vi "pvdf_forcereconstructor.vi"() -> ()   [LabVIEW 2023]
uses:
  MessageType.ctl
  <vilib>/Instr/_visa.llb/VISA Configure Serial Port (Instr).vi
panel:
  in  "?":enum32{"PVDF Plot", "Force Plot", "Heatmap"}(tab)
  out "Sensors data":T1(graph)
  out "Reconstructed force":T1(graph)
  out "Index":T2={"S2"=655360, "S3"=655360, "S6"=655360, "S7 3"=655360, "S8 4"=655360, "S4 2"=655360, "S1"=655360, "S5"=655360}
  out "Thumb":T2
  in  "?":T3(tab)
  in  "Header":string="<>\u0000"
  in  "Alpha":dbl=1.0 min=0.0 max=1.0
  out "READ BUFFER":string
  in  "COM_IE":refnum<visa-resource-name>="COM3"
  in  "Commands":string[](array[string])
  out "Error Out":errorcluster
  in  "Number of sensors":u32=16
  in  "block size":u32=100
  in  "PVDF Folder to Save":string="pvdf_data"
  in  "PVDF File Name Root":string="pvdf"
  out "Resulting pvdf saving path":path
  in  "Save pvdf only":bool
  in  "PVDF and Force Folder to Save":string="pvdf_force_data"
  in  "PVDF and Force File Name Root":string="pvdf_force"
  out "Resulting pvdf and force saving path":path
  in  "Save pvdf and force":bool
  in  "Active channels":bool[][](array[boolean])
  out "bytes to read":u32
  in  "TCP cluster":cluster{"data":dbl[][], "timestamp":u32[]}
  in  "pvdf and force save cluster":cluster{"Controls":T4, "data":string}
  in  "pvdf plot cluster":T1
  in  "pvdf save cluster":cluster{"Controls":T4, "data":string}
  in  "Stop":bool
  # "1"
  # "0.5"
  # "0"
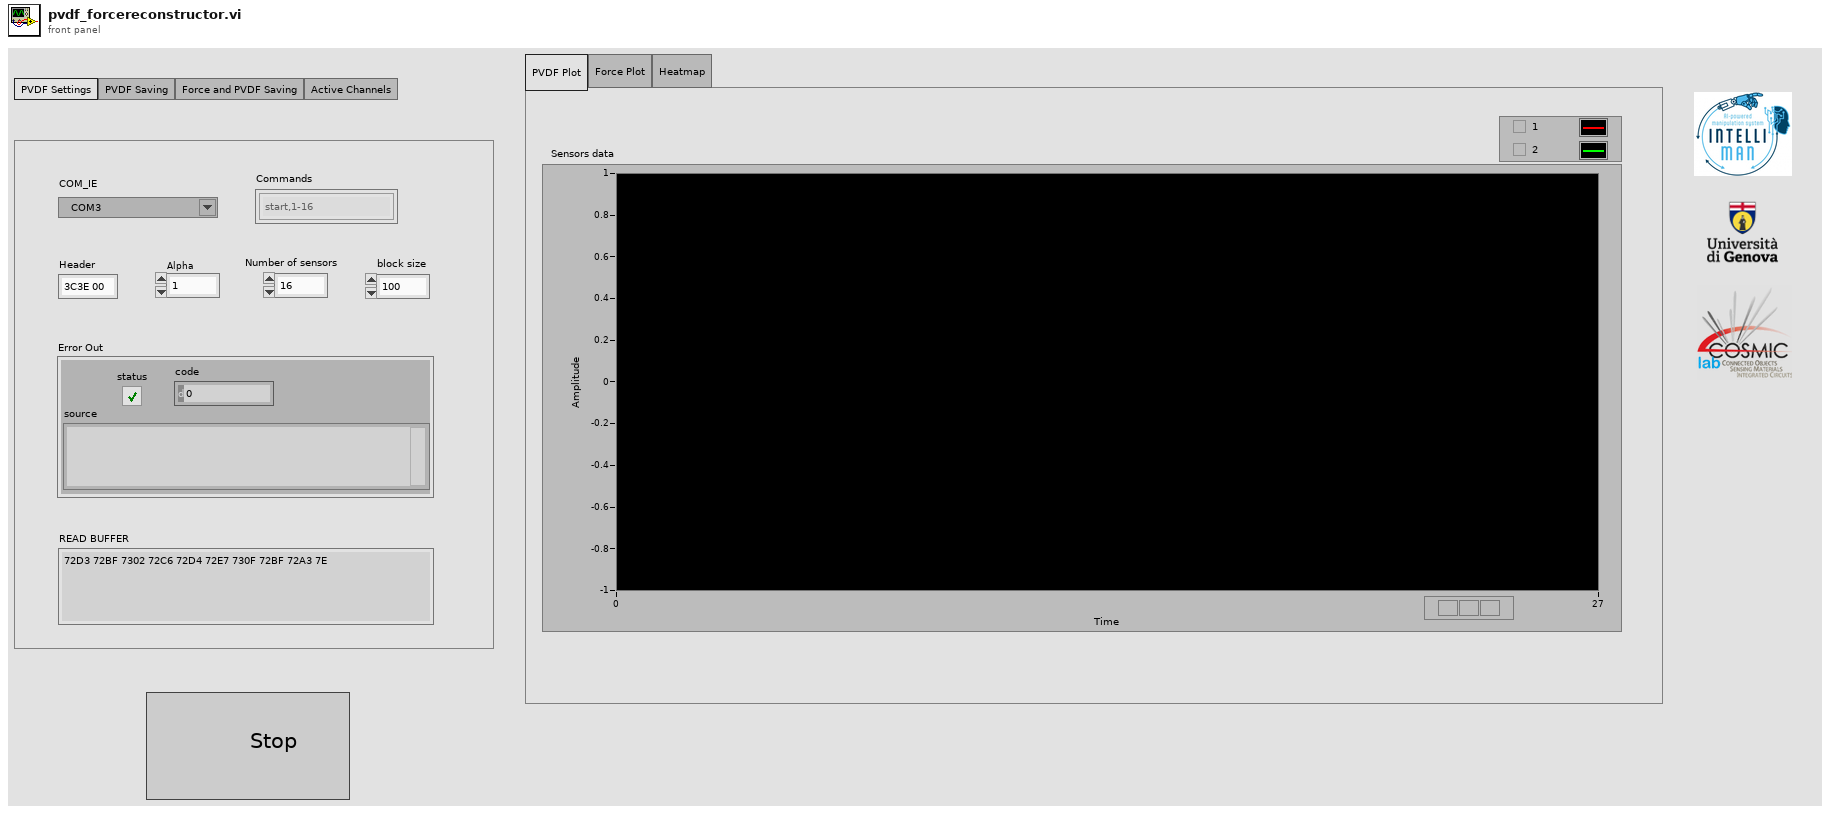
[diagram p1: front panel]
types:
  T1 = cluster{"[0]":dbl, "[1]":dbl, "[2]":dbl, "[3]":dbl, "[4]":dbl, "[5]":dbl, "[6]":dbl, "[7]":dbl, "[8]":dbl, "[9]":dbl, "[10]":dbl, "[11]":dbl, "[12]":dbl, "[13]":dbl, "[14]":dbl, "[15]":dbl, "[16]":dbl, "[17]":dbl, "[18]":dbl, "[19]":dbl, "[20]":dbl, "[21]":dbl, "[22]":dbl, "[23]":dbl, "[24]":dbl, "[25]":dbl, "[26]":dbl, "[27]":dbl, "[28]":dbl, "[29]":dbl, "[30]":dbl, "[31]":dbl, "[32]":dbl, "[33]":dbl, "[34]":dbl, "[35]":dbl, "[36]":dbl, "[37]":dbl, "[38]":dbl, "[39]":dbl, "[40]":dbl, "[41]":dbl, "[42]":dbl, "[43]":dbl, "[44]":dbl, "[45]":dbl, "[46]":dbl, "[47]":dbl, "[48]":dbl, "[49]":dbl, "[50]":dbl, "[51]":dbl, "[52]":dbl, "[53]":dbl, "[54]":dbl, "[55]":dbl, "[56]":dbl, "[57]":dbl, "[58]":dbl, "[59]":dbl, "[60]":dbl, "[61]":dbl, "[62]":dbl, "[63]":dbl}
  T2 = cluster{"S2":u32, "S3":u32, "S6":u32, "S7 3":u32, "S8 4":u32, "S4 2":u32, "S1":u32, "S5":u32}
  T3 = enum32{"PVDF Settings", "PVDF Saving", "Force and PVDF Saving", "Active Channels"}
  T4 = typedef "MessageType.ctl" = enum16{"data", "start_save", "stop_save", "active_channels"}
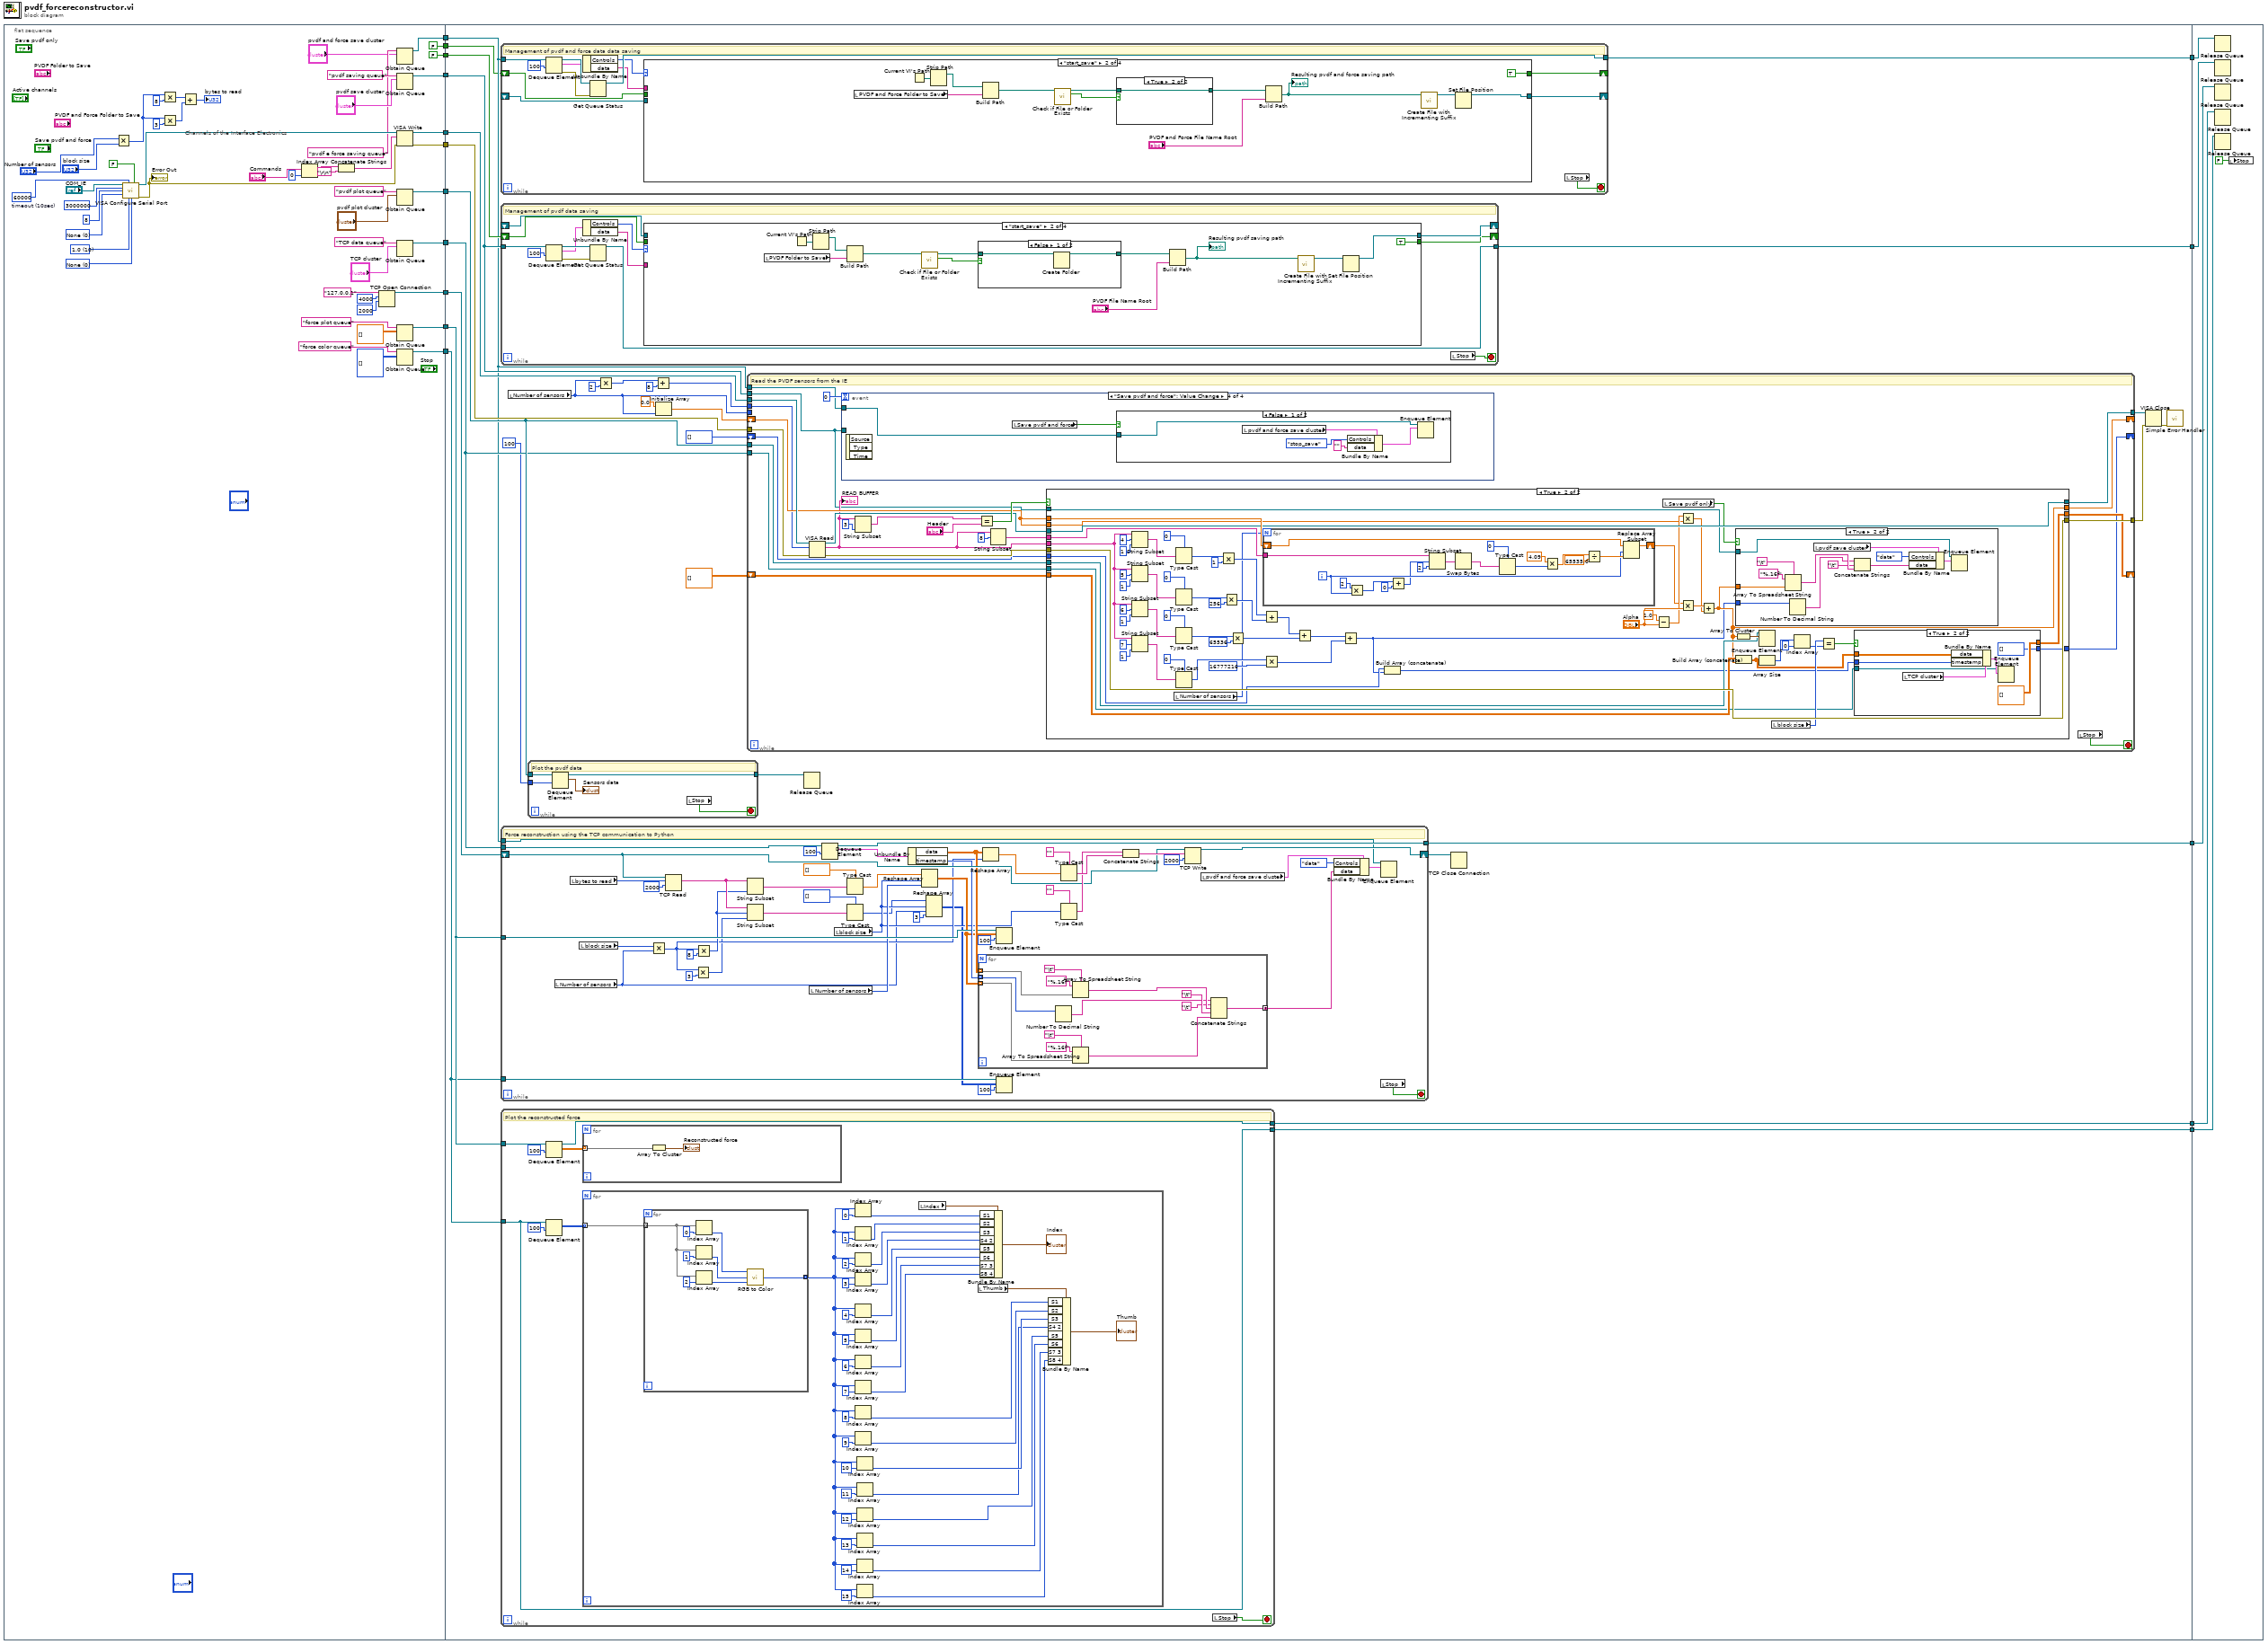
[diagram p0: block diagram]
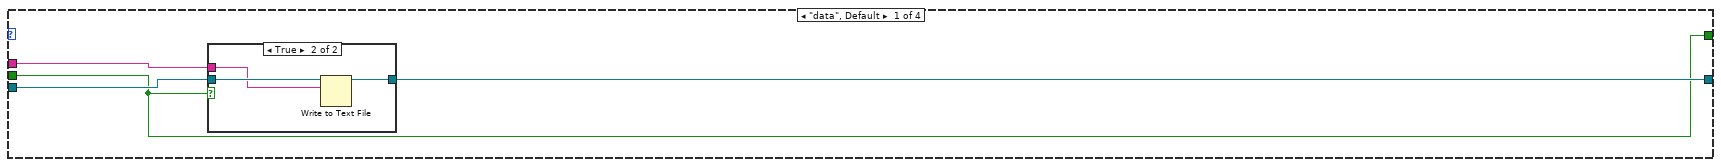
[diagram p2: hidden frame]
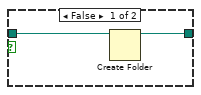
[diagram p4: hidden frame]
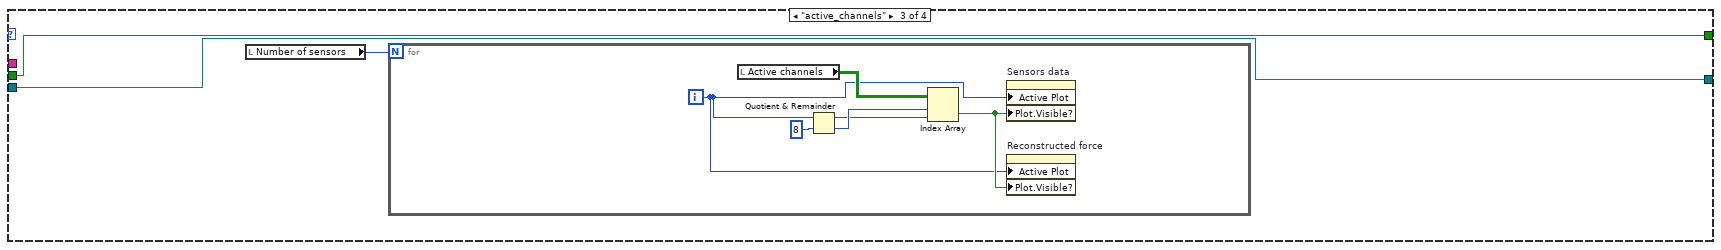
[diagram p5: hidden frame]
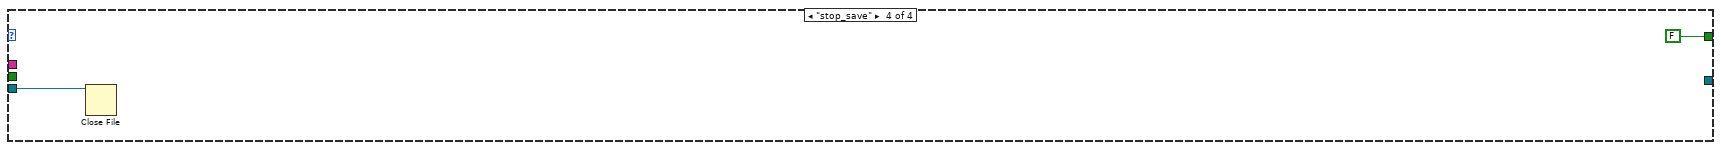
[diagram p6: hidden frame]
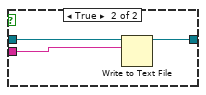
[diagram p8: hidden frame]
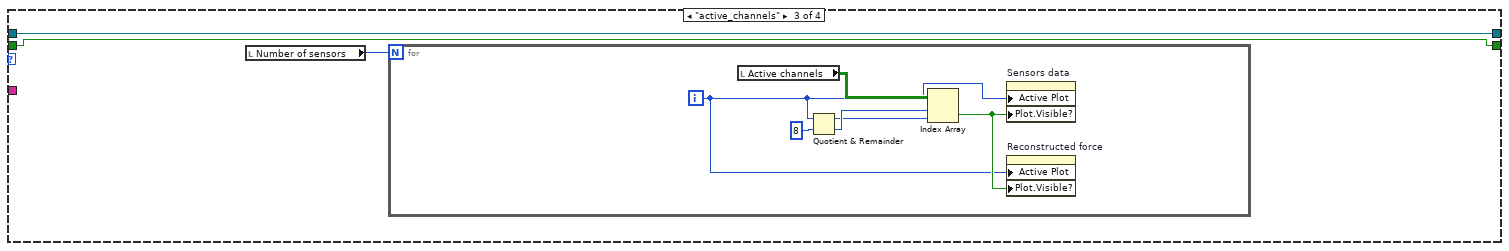
[diagram p10: hidden frame]
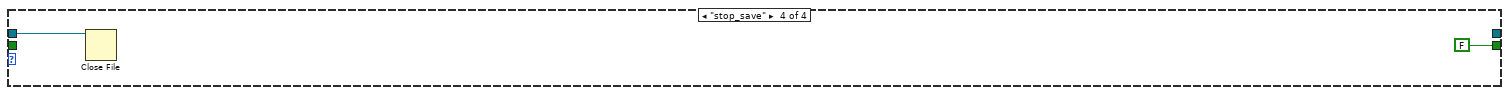
[diagram p11: hidden frame]
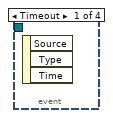
[diagram p12: hidden frame]
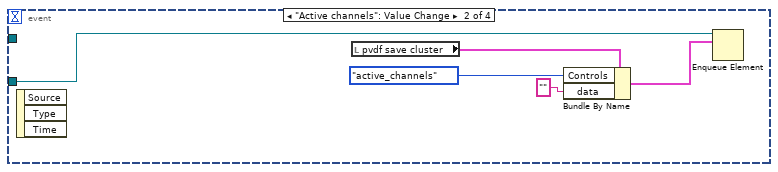
[diagram p13: hidden frame]
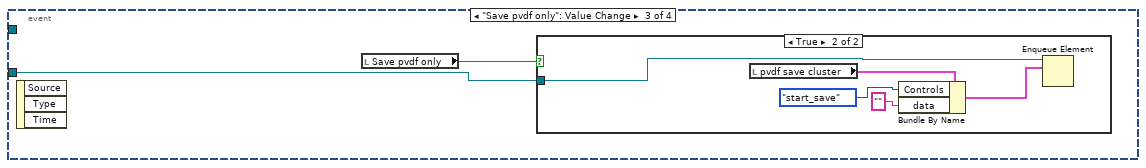
[diagram p14: hidden frame]
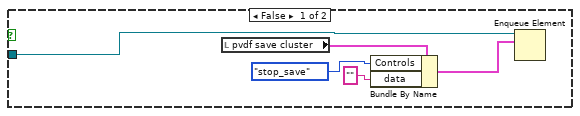
[diagram p15: hidden frame]
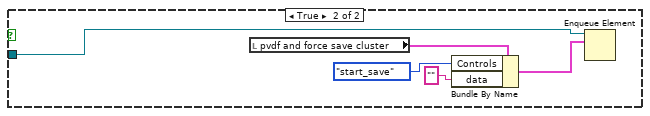
[diagram p16: hidden frame]
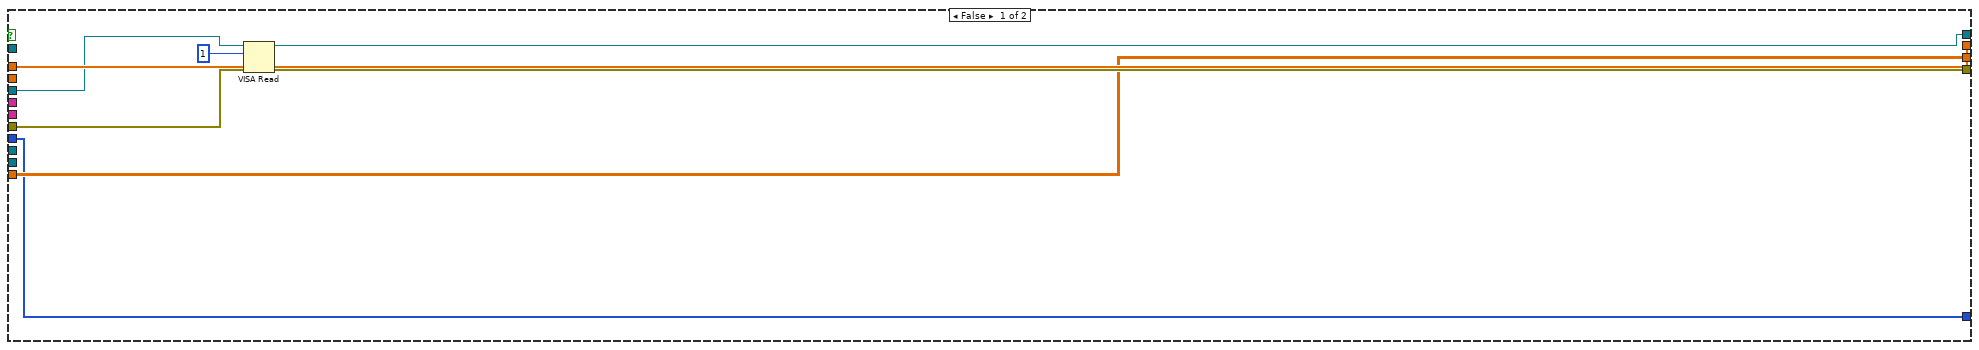
[diagram p17: hidden frame]
diagram:
  n1 = flat-sequence {
    tunnel: [w63] -> w16
    tunnel: [FALSE ("start save pvdf")] -> w15
    tunnel: [w60] -> w14
    tunnel: [w44] -> w13
    tunnel: [w43] -> w12
    tunnel: [w41] -> w11
    tunnel: [w38] -> w10
    tunnel: [w35] -> w9
    tunnel: [FALSE ("start save pvdf and force")] -> w8
    tunnel: [w29] -> w7
    tunnel: [w19] -> w6
    tunnel: w16 -> [w87]
    tunnel: w15 -> [w86]
    tunnel: w14 -> [w85]
    tunnel: w13 -> [w83]
    tunnel: w12 -> [w84]
    tunnel: w11 -> [w80]
    tunnel: w10 -> [w78]
    tunnel: w9 -> [w77]
    tunnel: w8 -> [w76]
    tunnel: w7 -> [w74]
    tunnel: w6 -> [w71]
    tunnel: [w70] -> w5
    tunnel: [w69] -> w4
    tunnel: [w68] -> w3
    tunnel: [w67] -> w2
    tunnel: [w66] -> w1
    tunnel: w5 -> [w477]
    tunnel: w4 -> [w476]
    tunnel: w3 -> [w475]
    tunnel: w2 -> [w474]
    tunnel: w1 -> [w473]
    frame #0 {
      w45 = u16 0 items=["None"=0, "XON/XOFF"=1, "RTS/CTS"=2, "DTR/DSR"=4] ("flow control")
      w51 = u32 60000  # timeout (10sec)
      w47 = u16 0 items=["None", "Odd", "Even", "Mark", "Space"] ("parity (0:none)")
      w46 = u16 10 items=["1.0"=10, "1.5"=15, "2.0"=20] ("stop bits")
      # "Channels of the Interface Electronics"
      n2 = Multiply(x="Number of sensors", y="block size") -> (x*y=w24:u32)
      n3 = call-poly "VISA Configure Serial Port"("VISA resource name"="COM_IE", "timeout (10sec)"=w51, "Enable Termination\nChar (T)"=FALSE ("Enable Termination\nChar (T)"), "baud rate (9600)"=u32 3000000, "data bits (8)"=u16 8, "parity (0:none)"=w47, "stop bits (10: 1 bit)"=w46, "flow control (0:none)"=w45) -> ("VISA resource name out"=w55:refnum<visa-resource-name>, "error out"=w56:errorcluster)  [unwired: 6 in]
      "Error Out" <- w56
      n4 = Multiply(x=w24, y=u32 8) -> (x*y=w26:u32)
      n5 = Multiply(x=w24, y=u32 3) -> (x*y=w25:u32)
      n6 = Add(x=w26, y=w25) -> (x+y=→"bytes to read":u32)
      n7 = Index Array(array="Commands", index=0) -> (element=w58:string)
      n8 = Concatenate Strings(w58, "\r\n") -> (w59:string)
      n9 = TCP Open Connection(address="127.0.0.1", remote port or service name=u16 4000, timeout ms (60000)=2000) -> (connection ID=w41:refnum<k5>)  [unwired: 2 in, 1 out]
      n10 = Obtain Queue(name (unnamed)="pvdf e force saving queue", element data type="pvdf and force save cluster") -> (queue out=w35:refnum<queue>)  [unwired: 3 in, 2 out]
      n11 = Obtain Queue(name (unnamed)="pvdf saving queue", element data type="pvdf save cluster") -> (queue out=w63:refnum<queue>)  [unwired: 3 in, 2 out]
      n12 = VISA Write(VISA resource name=w55, write buffer=w59, error in (no error)=w56) -> (VISA resource name out=w43:refnum<visa-resource-name>, error out=w44:errorcluster)  [unwired: 1 out]
      n13 = Obtain Queue(name (unnamed)="pvdf plot queue", element data type="pvdf plot cluster") -> (queue out=w60:refnum<queue>)  [unwired: 3 in, 2 out]
      n14 = Obtain Queue(name (unnamed)="TCP data queue", element data type="TCP cluster") -> (queue out=w38:refnum<queue>)  [unwired: 3 in, 2 out]
      n15 = Obtain Queue(name (unnamed)="force plot queue", element data type=dbl[][] []) -> (queue out=w29:refnum<queue>)  [unwired: 3 in, 2 out]
      n16 = Obtain Queue(name (unnamed)="force color queue", element data type=u8[][][] []) -> (queue out=w19:refnum<queue>)  [unwired: 3 in, 2 out]
    }
    frame #1 {
      n17 = while {
        tunnel: [w164] -> w68
        tunnel: w77 -> [w162]
        shift-right: [w159] -> _
        shift-left: _ -> [w156]
        shift-right: [w157] -> _
        shift-left: w76 -> [w158]
        stop <- w153 stop-if-true
        # "Management of pvdf and force data data saving"
        n18 = Dequeue Element(queue=w162, timeout in ms (-1)=100) -> (queue out=w165:refnum<queue>, element=w161:cluster{"Controls":T4, "data":string}, error out=w163:errorcluster)  [unwired: 1 in, 1 out]
        n19 = Unbundle By Name(w161) -> ("Controls"=w160:T4, "data"=w155:string)
        n20 = Get Queue Status(queue=w165, error in (no error)=w163) -> (queue out=w164:refnum<queue>)  [unwired: 1 in, 7 out]
        n21 = case shown="\"start_save\"" w160 {
          tunnel: [w167 w185 w190 _] -> w159
          tunnel: w158 -> [w166 _ w189 _]
          tunnel: [w166 TRUE w189 FALSE] -> w157
          tunnel: w156 -> [w168 _ w190 w198]
          tunnel: w155 -> [w169 _ _ _]
          frame "data", Default {
            n22 = case shown="True" w166 {
              tunnel: w169 -> [_ w172]
              tunnel: w168 -> [w170 w173]
              tunnel: [w170 w171] -> w167
              frame False {
              }
              frame True {
                n23 = Write to Text File(file (use dialog)=w173, text=w172) -> (refnum out=w171:refnum<file>)  [unwired: 2 in, 2 out]
              }
            }
          }
          frame "start_save" {
            n24 = local read "PVDF and Force Folder to Save"() -> (w181:string)
            n25 = Current VI's Path() -> (path=w183:path)
            n26 = Strip Path(path=w183) -> (stripped path=w182:path)  [unwired: 1 out]
            n27 = Build Path(base path=w182, name or relative path=w181) -> (appended path=w180:path)
            n28 = call <vilib>:"Check if File or Folder Exists.vi"("path"=w180) -> ("file or folder exists?"=w179:bool, "dup path"=w176:path)  [unwired: 8 in, 1 out]
            n29 = case shown="True" w179 {
              tunnel: [w187 w188] -> w177
              tunnel: w176 -> [w186 w188]
              frame False {
                n30 = Create Folder(path (use dialog)=w186) -> (created path=w187:path)  [unwired: 2 in, 2 out]
              }
              frame True {
              }
            }
            n31 = Build Path(base path=w177, name or relative path="PVDF and Force File Name Root") -> (appended path=w174:path)
            "Resulting pvdf and force saving path" <- w174
            n32 = call <vilib>:"Create File with Incrementing Suffix.vi"("file path"=w174) -> ("refnum out"=w178:refnum<file>)  [unwired: 8 in, 2 out]
            n33 = Set File Position(refnum=w178) -> (refnum out=w185:refnum<file>)  [unwired: 3 in, 1 out]
          }
          frame "active_channels" {
            n34 = local read "Number of sensors"() -> (w191:u32)
            n35 = for {
              N: w191 -> [_]
              i -> [w192]
              n36 = local read "Active channels"() -> (w197:bool[][])
              n37 = Quotient & Remainder(x=w192, y=8) -> (x-y*floor(x/y)=w194:i32, floor(x/y)=w195:i32)
              n38 = Index Array(array=w197, index (row)=w195, index (col)=w194) -> (element=w193:bool)
              n39 = property on="Sensors data" class="WFChart (strict)"("Active Plot"=w192, "Plot.Visible?"=w193) -> ()  [unwired: 2 in, 2 out]
              n40 = property on="Reconstructed force" class="WFChart (strict)"("Active Plot"=w192, "Plot.Visible?"=w193) -> ()  [unwired: 2 in, 2 out]
            }
          }
          frame "stop_save" {
            n41 = Close File(refnum=w198) -> ()  [unwired: 1 in, 2 out]
          }
        }
        n42 = local read "Stop"() -> (w153:bool)
      }
      n43 = while {
        tunnel: [w275] -> w66
        tunnel: w87 -> [w273]
        shift-right: [w270] -> _
        shift-left: _ -> [w267]
        shift-right: [w268] -> _
        shift-left: w86 -> [w269]
        stop <- w264 stop-if-true
        # "Management of pvdf data saving"
        n44 = Dequeue Element(queue=w273, timeout in ms (-1)=100) -> (queue out=w276:refnum<queue>, element=w272:cluster{"Controls":T4, "data":string}, error out=w274:errorcluster)  [unwired: 1 in, 1 out]
        n45 = Unbundle By Name(w272) -> ("Controls"=w271:T4, "data"=w266:string)
        n46 = Get Queue Status(queue=w276, error in (no error)=w274) -> (queue out=w275:refnum<queue>)  [unwired: 1 in, 7 out]
        n47 = case shown="\"start_save\"" w271 {
          tunnel: [w278 w285 w301 _] -> w270
          tunnel: w269 -> [w277 _ w300 _]
          tunnel: [w277 TRUE w300 FALSE] -> w268
          tunnel: w267 -> [w279 _ w301 w309]
          tunnel: w266 -> [w280 _ _ _]
          frame "data", Default {
            n48 = case shown="False" w277 {
              tunnel: w280 -> [_ w283]
              tunnel: w279 -> [w281 w284]
              tunnel: [w281 w282] -> w278
              frame False {
              }
              frame True {
                n49 = Write to Text File(file (use dialog)=w284, text=w283) -> (refnum out=w282:refnum<file>)  [unwired: 2 in, 2 out]
              }
            }
          }
          frame "start_save" {
            n50 = local read "PVDF Folder to Save"() -> (w294:string)
            n51 = Current VI's Path() -> (path=w292:path)
            n52 = Strip Path(path=w292) -> (stripped path=w293:path)  [unwired: 1 out]
            n53 = Build Path(base path=w293, name or relative path=w294) -> (appended path=w295:path)
            n54 = call <vilib>:"Check if File or Folder Exists.vi"("path"=w295) -> ("file or folder exists?"=w291:bool, "dup path"=w290:path)  [unwired: 8 in, 1 out]
            n55 = case shown="False" w291 {
              tunnel: [w298 w299] -> w286
              tunnel: w290 -> [w297 w299]
              frame False {
                n56 = Create Folder(path (use dialog)=w297) -> (created path=w298:path)  [unwired: 2 in, 2 out]
              }
              frame True {
              }
            }
            n57 = Build Path(base path=w286, name or relative path="PVDF File Name Root") -> (appended path=w289:path)
            "Resulting pvdf saving path" <- w289
            n58 = call <vilib>:"Create File with Incrementing Suffix.vi"("file path"=w289) -> ("refnum out"=w287:refnum<file>)  [unwired: 8 in, 2 out]
            n59 = Set File Position(refnum=w287) -> (refnum out=w285:refnum<file>)  [unwired: 3 in, 1 out]
          }
          frame "active_channels" {
            n60 = local read "Number of sensors"() -> (w302:u32)
            n61 = for {
              N: w302 -> [_]
              i -> [w303]
              n62 = local read "Active channels"() -> (w308:bool[][])
              n63 = Quotient & Remainder(x=w303, y=8) -> (x-y*floor(x/y)=w305:i32, floor(x/y)=w306:i32)
              n64 = Index Array(array=w308, index (row)=w306, index (col)=w305) -> (element=w304:bool)
              n65 = property on="Sensors data" class="WFChart (strict)"("Active Plot"=w303, "Plot.Visible?"=w304) -> ()  [unwired: 2 in, 2 out]
              n66 = property on="Reconstructed force" class="WFChart (strict)"("Active Plot"=w303, "Plot.Visible?"=w304) -> ()  [unwired: 2 in, 2 out]
            }
          }
          frame "stop_save" {
            n67 = Close File(refnum=w309) -> ()  [unwired: 1 in, 2 out]
          }
        }
        n68 = local read "Stop"() -> (w264:bool)
      }
      n69 = while {
        shift-right: [w235] -> w79
        shift-left: w80 -> [w234]
        tunnel: [w236] -> w67
        tunnel: w78 -> [w237]
        tunnel: w77 -> [w230]
        tunnel: w74 -> [w222]
        tunnel: w71 -> [w203]
        stop <- w220 stop-if-true
        # "Force reconstruction using the TCP communication to Python"
        n70 = local read "Number of sensors"() -> (w205:u32)
        n71 = local read "bytes to read"() -> (w219:u32)
        n72 = local read "block size"() -> (w217:u32)
        n73 = Multiply(x=w217, y=w205) -> (x*y=w212:u32)
        n74 = TCP Read(connection ID=w234, bytes to read=w219, 9:2000 ("timeout ms (25000)")) -> (data out=w214:string)  [unwired: 2 in, 2 out]
        n75 = Multiply(x=w212, y=u32 3) -> (x*y=w210:u32)
        n76 = Multiply(x=w212, y=u32 8) -> (x*y=w213:u32)
        n77 = String Subset(string=w214, length (rest)=w213) -> (substring=w216:string)  [unwired: 1 in]
        n78 = String Subset(string=w214, offset (0)=w213, length (rest)=w210) -> (substring=w209:string)
        n79 = local read "Number of sensors"() -> (w218:u32)
        n80 = Dequeue Element(queue=w237, timeout in ms (-1)=100) -> (queue out=w236:refnum<queue>, element=w226:cluster{"data":dbl[][], "timestamp":u32[]})  [unwired: 1 in, 2 out]
        n81 = local read "block size"() -> (w207:u32)
        n82 = Type Cast(type=dbl[] [], x=w216) -> (*(type *) &x=w244:dbl[])
        n83 = Type Cast(type=u8[] [], x=w209) -> (*(type *) &x=w206:u8[])
        n84 = Unbundle By Name(w226) -> ("data"=w225:dbl[][], "timestamp"=w224:u32[])
        n85 = Reshape Array(w244, w207, w218) -> (w221:dbl[][])
        n86 = Reshape Array(w206, w207, w205, 3 ("dimension size")) -> (w202:u8[][][])
        n87 = for {
          tunnel: w225 -> [w253] mode=indexing
          tunnel: w221 -> [w252] mode=indexing
          tunnel: [w249] -> w223 mode=concatenating
          tunnel: w224 -> [w248] mode=indexing
          n88 = Number To Decimal String(number=w248) -> (decimal integer string=w247:string)  [unwired: 1 in]
          n89 = Array To Spreadsheet String(delimiter (Tab)="\t", array=w253, 3:"%.16f" ("format string")) -> (spreadsheet string=w251:string)
          n90 = Array To Spreadsheet String(delimiter (Tab)="\t", array=w252, 3:"%.16f" ("format string")) -> (spreadsheet string=w258:string)
          n91 = Concatenate Strings(w247, "\t", w251, "\t", w258) -> (w249:string)
        }
        n92 = Reshape Array(w225, w212) -> (w239:dbl[])
        n93 = Enqueue Element(queue=w222, element=w221, timeout in ms (-1)=100) -> ()  [unwired: 1 in, 3 out]
        n94 = Enqueue Element(queue=w203, element=w202, timeout in ms (-1)=100) -> ()  [unwired: 1 in, 3 out]
        n95 = Type Cast(type="", x=w239) -> (*(type *) &x=w242:string)
        n96 = Type Cast(type="", x=w207) -> (*(type *) &x=w241:string)
        n97 = Concatenate Strings(w241, w242) -> (w243:string)
        n98 = TCP Write(connection ID=w234, data in=w243, 9:2000 ("timeout ms (25000)")) -> (connection ID out=w235:refnum<k5>)  [unwired: 1 in, 2 out]
        n99 = local read "pvdf and force save cluster"() -> (w229:cluster{"Controls":T4, "data":string})
        n100 = Bundle By Name(cluster=w229, "Controls"=MessageType."data", "data"=w223) -> (w228:cluster{"Controls":T4, "data":string})
        n101 = Enqueue Element(queue=w230, element=w228) -> ()  [unwired: 2 in, 3 out]
        n102 = local read "Stop"() -> (w220:bool)
      }
      n103 = while {
        tunnel: w74 -> [w104]
        tunnel: [w101] -> w69
        tunnel: w71 -> [w97]
        tunnel: [w97] -> w70
        stop <- w103 stop-if-true
        # "Plot the reconstructed force"
        n104 = Dequeue Element(queue=w104, timeout in ms (-1)=100) -> (queue out=w101:refnum<queue>, element=w100:dbl[][])  [unwired: 1 in, 2 out]
        n105 = Dequeue Element(queue=w97, timeout in ms (-1)=100) -> (element=w99:u8[][][])  [unwired: 1 in, 3 out]
        n106 = for {
          tunnel: w100 -> [w152] mode=indexing
          n107 = Array To Cluster(array=w152) -> (cluster=→"Reconstructed force":T1)
        }
        n108 = for {
          tunnel: w99 -> [w125] mode=indexing
          n109 = for {
            tunnel: w125 -> [w147] mode=indexing
            tunnel: [w150] -> w114 mode=indexing
            n110 = Index Array(array=w147, index=0) -> (element=w148:u8)
            n111 = Index Array(array=w147, index=1) -> (element=w144:u8)
            n112 = Index Array(array=w147, index=2) -> (element=w143:u8)
            n113 = call <vilib>:"RGB to Color.vi"("B"=w143, "G"=w144, "R"=w148) -> ("Color"=w150:u32)
          }
          n114 = Index Array(array=w114, index=0) -> (element=w139:u32)
          n115 = Index Array(array=w114, index=1) -> (element=w107:u32)
          n116 = Index Array(array=w114, index=2) -> (element=w138:u32)
          n117 = Index Array(array=w114, index=3) -> (element=w136:u32)
          n118 = Index Array(array=w114, index=4) -> (element=w135:u32)
          n119 = Index Array(array=w114, index=5) -> (element=w134:u32)
          n120 = Index Array(array=w114, index=6) -> (element=w133:u32)
          n121 = Index Array(array=w114, index=7) -> (element=w132:u32)
          n122 = Index Array(array=w114, index=8) -> (element=w113:u32)
          n123 = Index Array(array=w114, index=9) -> (element=w112:u32)
          n124 = Index Array(array=w114, index=10) -> (element=w111:u32)
          n125 = Index Array(array=w114, index=11) -> (element=w106:u32)
          n126 = Index Array(array=w114, index=12) -> (element=w105:u32)
          n127 = Index Array(array=w114, index=13) -> (element=w110:u32)
          n128 = Index Array(array=w114, index=14) -> (element=w109:u32)
          n129 = Index Array(array=w114, index=15) -> (element=w108:u32)
          n130 = local read "Index"() -> (w142:T2)
          n131 = local read "Thumb"() -> (w124:T2)
          n132 = Bundle By Name(cluster=w142, "S1"=w139, "S2"=w107, "S3"=w138, "S4 2"=w136, "S5"=w135, "S6"=w134, "S7 3"=w133, "S8 4"=w132) -> (→"Index":T2)
          n133 = Bundle By Name(cluster=w124, "S1"=w113, "S2"=w112, "S3"=w111, "S4 2"=w106, "S5"=w105, "S6"=w110, "S7 3"=w109, "S8 4"=w108) -> (→"Thumb":T2)
        }
        n134 = local read "Stop"() -> (w103:bool)
      }
      n135 = local read "Number of sensors"() -> (w73:u32)
      n136 = while {
        tunnel: w85 -> [w263]
        tunnel: [w261] -> w81
        tunnel: 100 ("timeout in ms (-1)") -> [w259]
        stop <- w260 stop-if-true
        # "Plot the pvdf data"
        n137 = Dequeue Element(queue=w263, timeout in ms (-1)=w259) -> (queue out=w261:refnum<queue>, element=→"Sensors data":T1)  [unwired: 1 in, 2 out]
        n138 = local read "Stop"() -> (w260:bool)
      }
      n139 = Multiply(x=w73, y=2) -> (x*y=w89:u32)
      n140 = Add(x=w89, y=8) -> (x+y=w88:u32)
      n141 = Initialize Array(0.0, w73) -> (w95:dbl[])
      n142 = while {
        shift-right: [w336] -> _
        shift-left: w95 -> [w325]
        tunnel: w83 -> [w335]
        tunnel: w84 -> [w334]
        tunnel: [w328] -> w92
        tunnel: [w327] -> w93
        tunnel: w73 -> [_]
        tunnel: w88 -> [w321]
        tunnel: w87 -> [w318]
        tunnel: w85 -> [w317]
        shift-right: [w315] -> _
        shift-left: dbl[][] [] -> [w316]
        tunnel: w78 -> [w314]
        tunnel: w77 -> [w313]
        shift-right: [w311] -> _
        shift-left: u32[] [] -> [w312]
        stop <- w319 stop-if-true
        # "Read the PVDF sensors from the IE"
        n143 = VISA Read(VISA resource name=w334, byte count=w321, error in (no error)=w335) -> (VISA resource name out=w330:refnum<visa-resource-name>, read buffer=w322:string, error out=w329:errorcluster)  [unwired: 1 out]
        "READ BUFFER" <- w322
        n144 = event shown="[3] \"Save pvdf and force\": Value Change" {
          selector: _ -> [_ _ _ _]
          dyn-events: _ -> [_ _ _ _]
          timeout: 0 -> [_ _ _ _]
          tunnel: w318 -> [_ w341 w342 _]
          tunnel: w313 -> [_ _ _ w354]
          event Timeout {
            n145 = event-data() -> ()  [unwired: 1 in, 3 out]
          }
          event "Active channels": Value Change {
            n146 = event-data() -> ()  [unwired: 1 in, 3 out]
            n147 = local read "pvdf save cluster"() -> (w340:cluster{"Controls":T4, "data":string})
            n148 = Bundle By Name(cluster=w340, "Controls"=MessageType."active_channels" ("Enum"), "data"="") -> (w338:cluster{"Controls":T4, "data":string})
            n149 = Enqueue Element(queue=w341, element=w338) -> ()  [unwired: 2 in, 3 out]
          }
          event "Save pvdf only": Value Change {
            n150 = event-data() -> ()  [unwired: 1 in, 3 out]
            n151 = local read "Save pvdf only"() -> (w343:bool)
            n152 = case shown="True" w343 {
              tunnel: w342 -> [w348 w351]
              frame False {
                n153 = local read "pvdf save cluster"() -> (w347:cluster{"Controls":T4, "data":string})
                n154 = Bundle By Name(cluster=w347, "Controls"=MessageType."stop_save" ("Enum"), "data"="") -> (w346:cluster{"Controls":T4, "data":string})
                n155 = Enqueue Element(queue=w348, element=w346) -> ()  [unwired: 2 in, 3 out]
              }
              frame True {
                n156 = local read "pvdf save cluster"() -> (w353:cluster{"Controls":T4, "data":string})
                n157 = Bundle By Name(cluster=w353, "Controls"=MessageType."start_save" ("Enum"), "data"="") -> (w350:cluster{"Controls":T4, "data":string})
                n158 = Enqueue Element(queue=w351, element=w350) -> ()  [unwired: 2 in, 3 out]
              }
            }
          }
          event "Save pvdf and force": Value Change {
            n159 = event-data() -> ()  [unwired: 1 in, 3 out]
            n160 = local read "Save pvdf and force"() -> (w355:bool)
            n161 = case shown="False" w355 {
              tunnel: w354 -> [w360 w365]
              frame False {
                n162 = local read "pvdf and force save cluster"() -> (w358:cluster{"Controls":T4, "data":string})
                n163 = Bundle By Name(cluster=w358, "Controls"=MessageType."stop_save", "data"="") -> (w356:cluster{"Controls":T4, "data":string})
                n164 = Enqueue Element(queue=w360, element=w356) -> ()  [unwired: 2 in, 3 out]
              }
              frame True {
                n165 = local read "pvdf and force save cluster"() -> (w363:cluster{"Controls":T4, "data":string})
                n166 = Bundle By Name(cluster=w363, "Controls"=MessageType."start_save", "data"="") -> (w361:cluster{"Controls":T4, "data":string})
                n167 = Enqueue Element(queue=w365, element=w361) -> ()  [unwired: 2 in, 3 out]
              }
            }
          }
        }
        n168 = String Subset(string=w322, length (rest)=3 ("length (rest)")) -> (substring=w332:string)  [unwired: 1 in]
        n169 = Equal?(x=w332, y="Header") -> (x = y?=w333:bool)
        n170 = String Subset(string=w322, offset (0)=8) -> (substring=w324:string)  [unwired: 1 in]
        n171 = case shown="True" w333 {
          tunnel: w325 -> [w373 w434]
          tunnel: [w373 w387] -> w336
          tunnel: w324 -> [_ w433]
          tunnel: w330 -> [w372 w432]
          tunnel: w329 -> [w371 w431]
          tunnel: [w369 w432] -> w328
          tunnel: [w368 w431] -> w327
          tunnel: w325 -> [_ w424]
          tunnel: w322 -> [_ w404]
          tunnel: w318 -> [_ w391]
          tunnel: w317 -> [_ w389]
          tunnel: w316 -> [w367 w388]
          tunnel: [w367 w381] -> w315
          tunnel: w314 -> [_ w379]
          tunnel: w312 -> [w366 w378]
          tunnel: [w366 w375] -> w311
          frame False {
            n172 = VISA Read(VISA resource name=w372, byte count=u32 1, error in (no error)=w371) -> (VISA resource name out=w369:refnum<visa-resource-name>, error out=w368:errorcluster)  [unwired: 2 out]
          }
          frame True {
            n173 = String Subset(string=w404, offset (0)=4, length (rest)=1 ("length (rest)")) -> (substring=w418:string)
            n174 = String Subset(string=w404, offset (0)=5, length (rest)=1 ("length (rest)")) -> (substring=w412:string)
            n175 = String Subset(string=w404, offset (0)=6, length (rest)=1 ("length (rest)")) -> (substring=w410:string)
            n176 = String Subset(string=w404, offset (0)=7, length (rest)=1 ("length (rest)")) -> (substring=w408:string)
            n177 = local read "Number of sensors"() -> (w374:u32)
            n178 = Type Cast(type=u8 0, x=w418) -> (*(type *) &x=w403:u8)
            n179 = Type Cast(type=u8 0, x=w412) -> (*(type *) &x=w405:u8)
            n180 = Type Cast(type=u8 0, x=w410) -> (*(type *) &x=w406:u8)
            n181 = Type Cast(type=u8 0, x=w408) -> (*(type *) &x=w407:u8)
            n182 = Multiply(x=w403, y=u32 1) -> (x*y=w398:u32)
            n183 = Multiply(x=w405, y=u32 256) -> (x*y=w397:u32)
            n184 = Multiply(x=w406, y=u32 65536) -> (x*y=w395:u32)
            n185 = for {
              N: w374 -> [_]
              shift-right: [w469] -> w425
              shift-left: w434 -> [w468]
              tunnel: w433 -> [w463]
              i -> [w466]
              n186 = Multiply(x=2, y=w466) -> (x*y=w458:i32)
              n187 = Add(x=w458, y=0 ("offset (0)")) -> (x+y=w456:i32)
              n188 = String Subset(string=w463, offset (0)=w456, length (rest)=2 ("length (rest)")) -> (substring=w462:string)
              n189 = Swap Bytes(anything=w462) -> (byte swapped=w461:string)
              n190 = Type Cast(type=u16 0, x=w461) -> (*(type *) &x=w459:u16)
              n191 = Multiply(x=4.09 ("y"), y=w459) -> (x*y=w470:dbl)
              n192 = Divide(x=w470, y=65535.0) -> (x/y=w467:dbl)
              n193 = Replace Array Subset(array=w468, new element=w467, index=w466) -> (w469:dbl[])
            }
            n194 = Add(x=w398, y=w397) -> (x+y=w396:u32)
            n195 = Multiply(x=w407, y=u32 16777216) -> (x*y=w394:u32)
            n196 = Add(x=w396, y=w395) -> (x+y=w393:u32)
            n197 = Add(x=w393, y=w394) -> (x+y=w377:u32)
            n198 = Build Array (concatenate)(w378, w377) -> (w376:u32[])
            n199 = Subtract(x=1.0, y="Alpha") -> (x-y=w427:dbl)
            n200 = local read "Save pvdf only"() -> (w392:bool)
            n201 = Multiply(x=w427, y=w424) -> (x*y=w426:dbl[])
            n202 = Multiply(x=w425, y="Alpha") -> (x*y=w430:dbl[])
            n203 = Add(x=w430, y=w426) -> (x+y=w387:dbl[])
            n204 = Array To Cluster(array=w387) -> (cluster=w390:T1)
            n205 = case shown="True" w392 {
              tunnel: w377 -> [_ w450]
              tunnel: w387 -> [_ w449]
              tunnel: w391 -> [_ w447]
              frame False {
              }
              frame True {
                n206 = Array To Spreadsheet String(delimiter (Tab)="\t", array=w449, 3:"%.16f" ("format string")) -> (spreadsheet string=w455:string)
                n207 = Number To Decimal String(number=w450) -> (decimal integer string=w454:string)  [unwired: 1 in]
                n208 = local read "pvdf save cluster"() -> (w445:cluster{"Controls":T4, "data":string})
                n209 = Concatenate Strings(w454, "\t", w455) -> (w444:string)
                n210 = Bundle By Name(cluster=w445, "Controls"=MessageType."data" ("Enum"), "data"=w444) -> (w446:cluster{"Controls":T4, "data":string})
                n211 = Enqueue Element(queue=w447, element=w446) -> ()  [unwired: 2 in, 3 out]
              }
            }
            n212 = Build Array (concatenate)(w388, w387) -> (w380:dbl[][])
            n213 = Enqueue Element(queue=w389, element=w390) -> ()  [unwired: 2 in, 3 out]
            n214 = Array Size(array=w380) -> (size(s)=w386:i32[])
            n215 = local read "block size"() -> (w384:u32)
            n216 = Index Array(array=w386, index=0) -> (element=w383:i32)
            n217 = Equal?(x=w384, y=w383) -> (x = y?=w382:bool)
            n218 = case shown="True" w382 {
              tunnel: [w436 dbl[][] []] -> w381
              tunnel: w380 -> [w436 w441]
              tunnel: w379 -> [_ w437]
              tunnel: w376 -> [w435 w438]
              tunnel: [w435 u32[] []] -> w375
              frame False {
              }
              frame True {
                n219 = local read "TCP cluster"() -> (w442:cluster{"data":dbl[][], "timestamp":u32[]})
                n220 = Bundle By Name(cluster=w442, "data"=w441, "timestamp"=w438) -> (w440:cluster{"data":dbl[][], "timestamp":u32[]})
                n221 = Enqueue Element(queue=w437, element=w440) -> ()  [unwired: 2 in, 3 out]
              }
            }
          }
        }
        n222 = local read "Stop"() -> (w319:bool)
      }
      n223 = Release Queue(queue=w81) -> ()  [unwired: 2 in, 3 out]
      n224 = TCP Close Connection(connection ID=w79) -> ()  [unwired: 2 in, 2 out]
      n225 = VISA Close(VISA resource name=w92, error in (no error)=w93) -> (error out=w94:errorcluster)
      n226 = call <vilib>:"Simple Error Handler.vi"("error in (no error)"=w94) -> ()  [unwired: 1 in, 8 out]
    }
    frame #2 {
      n227 = Release Queue(queue=w475) -> ()  [unwired: 2 in, 3 out]
      n228 = Release Queue(queue=w473) -> ()  [unwired: 2 in, 3 out]
      n229 = Release Queue(queue=w474) -> ()  [unwired: 2 in, 3 out]
      n230 = Release Queue(queue=w476) -> ()  [unwired: 2 in, 3 out]
      n231 = Release Queue(queue=w477) -> ()  [unwired: 2 in, 3 out]
      n232 = local write "Stop"(FALSE ("stop all")) -> ()
    }
  }
